vi "linked-ignore.vi"(11 "error in":errorcluster) -> (15 "error out":errorcluster)   [LabVIEW 2024]
doc: "Data-only fixture for object-scoped hardcoded-secret-default ignores. All credential text is fictitious."
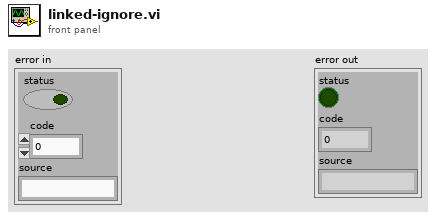
[diagram p1: front panel]
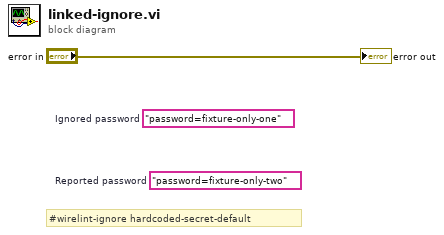
[diagram p0: block diagram]
diagram:
  (unwired) "password=fixture-only-two"  # Reported password
  (unwired) "password=fixture-only-one"  # Ignored password
  # "#wirelint-ignore hardcoded-secret-default"
  "error out" <- "error in"
